vi "[ce] INI - RW MCList Properties.vi"(6 "cmd (load)":enum16{"load", "save"}(ring), 8 "error in":errorcluster, 10 "MCListbox Refnum":refnum<vi>, 11 "INI refnum":T1) -> (0 "error out":errorcluster, 3 "dup INI refnum":T1)   [LabVIEW 2021]
doc: "::: CalcExpress Toolkit :::\nCopyright (c) 2000-2026 Konstantin Shifershteyn. All rights reserved."
uses:
  <vilib>/Utility/config.llb/Config Data RefNum.ctl
  <vilib>/Utility/config.llb/Read Key (U32).vi
  <vilib>/Utility/config.llb/Write Key (U32).vi
  <vilib>/Utility/config.llb/NI_LVConfig.lvlib
panel:
  out "Array":cluster{"Column":i32, "Width":u32}[](array[cluster])
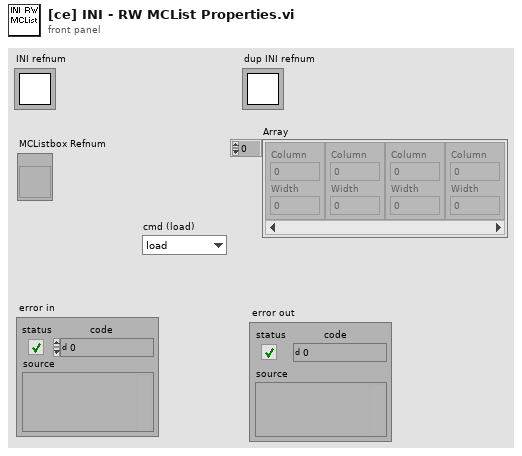
[diagram p1: front panel]
types:
  T1 = typedef "NI_LVConfig.lvlib/Config Data RefNum.ctl" = refnum<k1>
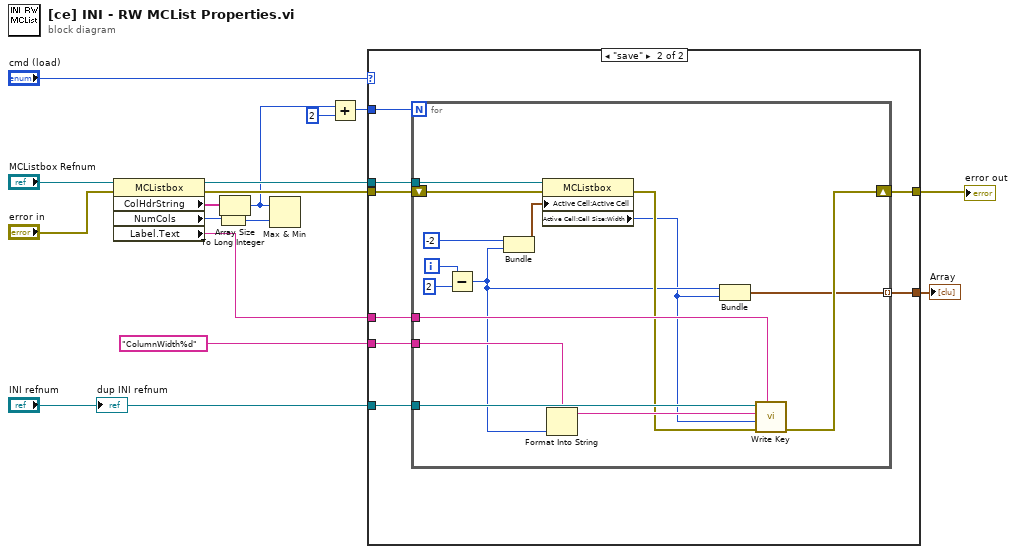
[diagram p0: block diagram]
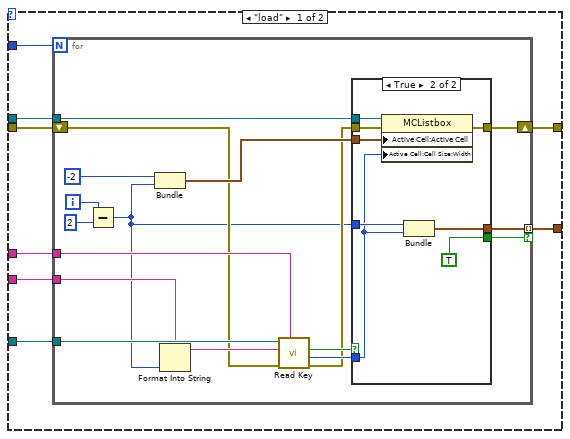
[diagram p2: hidden frame]
diagram:
  n1 = property class="MCListbox"(reference="MCListbox Refnum", error in="error in") -> (reference out=w13:refnum<vi>, error out=w12:errorcluster, "ColHdrString"=w15:string[], "NumCols"=w14:u32, "Label.Text"=w8:string)
  n2 = To Long Integer(number=w14) -> (32bit integer=w10:i32)
  n3 = Array Size(array=w15) -> (size(s)=w1:i32)
  n4 = Max & Min(x=w1, y=w10) -> ()  [unwired: 2 out]
  n5 = Add(x=w1, y=2) -> (x+y=w11:i32)
  n6 = case shown="\"save\"" "cmd (load)" {
    tunnel: w13 -> [w24 w58]
    tunnel: w12 -> [w23 w57]
    tunnel: w11 -> [w22 w56]
    tunnel: w8 -> [w21 w55]
    tunnel: "INI refnum" -> [w20 w54]
    tunnel: "ColumnWidth%d" ("format string") -> [w19 w53]
    tunnel: [w18 w52] -> w4
    tunnel: [w17 w51] -> w2
    frame "load" {
      n7 = for {
        N: w22 -> [_]
        tunnel: w24 -> [w41]
        shift-right: [w28] -> w18
        shift-left: w23 -> [w30]
        tunnel: w21 -> [w37]
        tunnel: w20 -> [w36]
        tunnel: w19 -> [w33]
        tunnel: [w26] -> w17 mode=indexing if=w25
        i -> [w40]
        n8 = Subtract(x=w40, y=2) -> (x-y=w27:i32)
        n9 = Bundle("Row"=-2, w27) -> (w38:cluster{"Row":i32, i32})  [unwired: 1 in]
        n10 = Format Into String(format string=w33, w27) -> (resulting string=w34:string)  [unwired: 2 in, 1 out]
        n11 = call-poly <vilib>:"Read Key.vi"("section"=w37, "error in (no error)"=w30, "key"=w34, "refnum"=w36) -> ("error out"=w29:errorcluster, "value"=w31:u32, "found?"=w32:bool)  [unwired: 4 in, 1 out]
        n12 = case shown="True" w32 {
          tunnel: w41 -> [_ w50]
          tunnel: w38 -> [_ w49]
          tunnel: w31 -> [_ w45]
          tunnel: w29 -> [w42 w48]
          tunnel: [w42 w47] -> w28
          tunnel: w27 -> [_ w46]
          tunnel: [_ w44] -> w26
          tunnel: [_ TRUE] -> w25
          frame False {
          }
          frame True {
            n13 = property class="MCListbox"(reference=w50, error in=w48, "Active Cell:Active Cell"=w49, "Active Cell:Cell Size:Width"=w45) -> (error out=w47:errorcluster)  [unwired: 1 out]
            n14 = Bundle(w46, "value"=w45) -> (w44:cluster{i32, "value":u32})  [unwired: 1 in]
          }
        }
      }
    }
    frame "save" {
      n15 = for {
        N: w56 -> [_]
        tunnel: w58 -> [w73]
        shift-right: [w62] -> w52
        shift-left: w57 -> [w70]
        tunnel: w55 -> [w68]
        tunnel: w54 -> [w67]
        tunnel: w53 -> [w64]
        tunnel: [w61] -> w51 mode=indexing
        i -> [w72]
        n16 = Subtract(x=w72, y=2) -> (x-y=w60:i32)
        n17 = Bundle("Row"=-2, w60) -> (w69:cluster{"Row":i32, i32})  [unwired: 1 in]
        n18 = property class="MCListbox"(reference=w73, error in=w70, "Active Cell:Active Cell"=w69) -> (error out=w63:errorcluster, "Active Cell:Cell Size:Width"=w59:u32)  [unwired: 1 out]
        n19 = Format Into String(format string=w64, w60) -> (resulting string=w65:string)  [unwired: 2 in, 1 out]
        n20 = Bundle(w60, "Width"=w59) -> (w61:cluster{i32, "Width":u32})  [unwired: 1 in]
        n21 = call-poly <vilib>:"Write Key.vi"("section"=w68, "error in (no error)"=w63, "value"=w59, "key"=w65, "refnum"=w67) -> ("error out"=w62:errorcluster)  [unwired: 4 in, 2 out]
      }
    }
  }
  "error out" <- w4
  "Array" <- w2
  "dup INI refnum" <- "INI refnum"
